vi "ZM-CP-init.vi"(8 "error in (no error)":errorcluster, 11 "ZM-CP-communication_protocol in":refnum<class "ZM-CP-communication_protocol.lvclass">) -> (0 "error out":errorcluster, 3 "ZM-CP-communication_protocol out":refnum<class "ZM-CP-communication_protocol.lvclass">)   [LabVIEW 2020, in "ZM-CP-communication_protocol.lvlib" / "ZM-CP-communication_protocol.lvclass"]
doc: "Initialises the communication protocol (dynamic dispatch): writes opened = TRUE through the private accessor Write opened. This is the real default of the parent; a child overrides it, calls the parent and then runs its own hook."
uses:
  ZM-CP-communication_protocol.lvclass
  ZM-CP-communication_protocol.lvclass/ZM-CP-communication_protocol.ctl
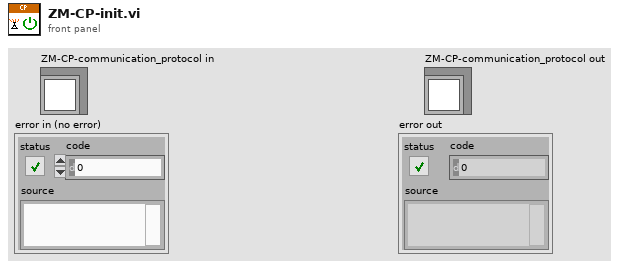
[diagram p1: front panel]
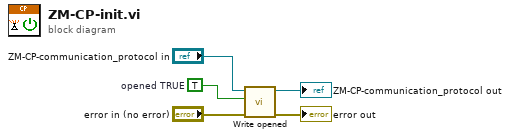
[diagram p0: block diagram]
diagram:
  w3 = TRUE  # opened TRUE
  n1 = call "Write opened.vi"("error in (no error)"="error in (no error)", "opened"=w3, "ZM-CP-communication_protocol in"="ZM-CP-communication_protocol in") -> ("error out"=→"error out":errorcluster, "ZM-CP-communication_protocol out"=→"ZM-CP-communication_protocol out":refnum<class "ZM-CP-communication_protocol.lvclass">)  [unwired: 7 in]
